vi "query OBW Measurement Result.vi"(8 "error in (no error)":errorcluster, 11 "Keysight 9020A in":refnum<class "Keysight 9020A.lvclass">) -> (0 "error out":errorcluster, 2 "OBW Measurement":T1, 3 "Keysight 9020A out":refnum<class "Keysight 9020A.lvclass">)   [LabVIEW 2023, in "Spectrum Analyzer.lvlib" / "Keysight 9020A.lvclass"]
uses:
  Keysight 9020A.lvclass
  TYPE DEFINITION/SA Measurement Class/TYPE OBW Measurement.ctl
  TYPE DEFINITION/TYPE query Data Processing Type.ctl
  Keysight 9020A.lvclass/Keysight 9020A.ctl
  Spectrum Analyzer.lvlib
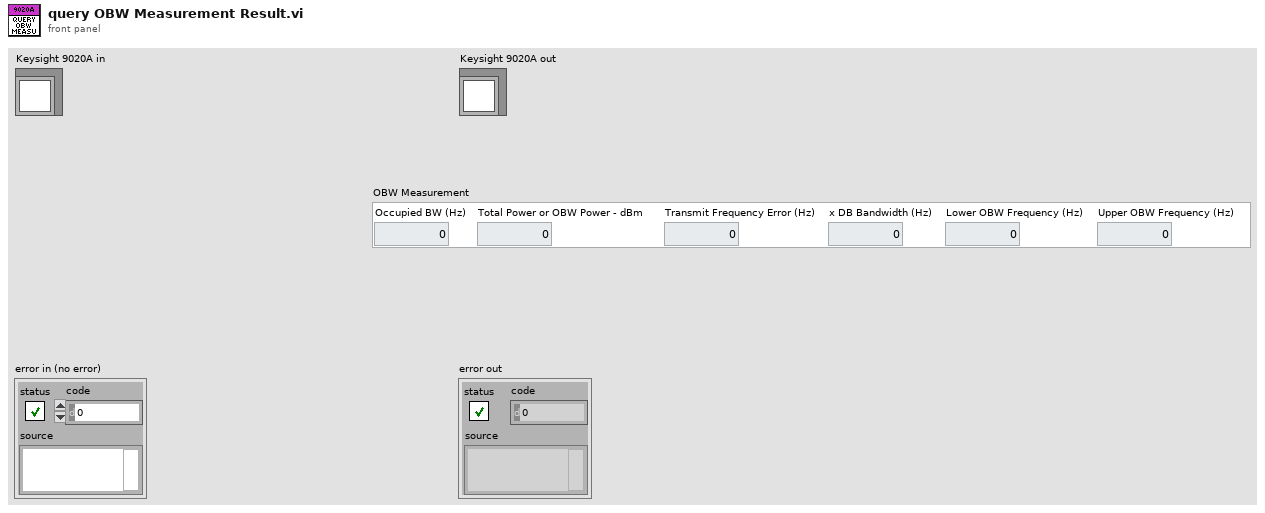
[diagram p1: front panel]
types:
  T1 = typedef "Spectrum Analyzer.lvlib/TYPE OBW Measurement.ctl" = cluster{"Occupied BW (Hz)":dbl, "Total Power or OBW Power - dBm":dbl, "Transmit Frequency Error (Hz)":dbl, "x DB Bandwidth (Hz)":dbl, "Lower OBW Frequency (Hz)":dbl, "Upper OBW Frequency (Hz)":dbl}
  T2 = typedef "Spectrum Analyzer.lvlib/TYPE query Data Processing Type.ctl" = enum16{"Fetch", "Measure", "Read"}
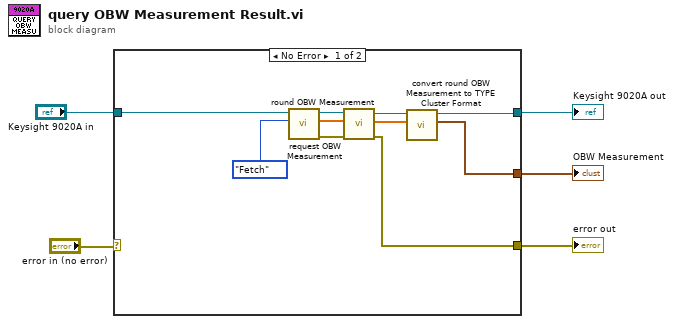
[diagram p0: block diagram]
diagram:
  n1 = case shown="No Error" "error in (no error)" {
    selector: "error in (no error)" -> [_ w16]
    tunnel: "Keysight 9020A in" -> [w15 w17]
    tunnel: [w8 w17] -> w4
    tunnel: [w10 w16] -> w2
    tunnel: [w6 _] -> w1
    frame No Error {
      n2 = call "request OBW Measurement.vi"("Query Mode"=TYPE_query_Data_Processing_Type."Fetch", "Keysight 9020A in"=w15) -> ("error out"=w12:errorcluster, "OBW Measurement Result Array"=w11:dbl[], "Keysight 9020A out"=w13:refnum<class "Keysight 9020A.lvclass">)  [unwired: 7 in]
      n3 = call "round OBW Measurement.vi"("error in (no error)"=w12, "OBW Measurement Raw Result"=w11, "Keysight 9020A in"=w13) -> ("error out"=w10:errorcluster, "OBW Measurement Rounded Result"=w7:dbl[], "Keysight 9020A out"=w9:refnum<class "Keysight 9020A.lvclass">)  [unwired: 6 in]
      n4 = call "convert round OBW Measurement to TYPE Cluster Format.vi"("OBW Measurement Rounded Result"=w7, "Keysight 9020A in"=w9) -> ("OBW Measurement"=w6:T1, "Keysight 9020A out"=w8:refnum<class "Keysight 9020A.lvclass">)  [unwired: 7 in, 1 out]
    }
    frame Error {
    }
  }
  "error out" <- w2
  "Keysight 9020A out" <- w4
  "OBW Measurement" <- w1
